vi "GCD and LCM.vi"() -> ()   [LabVIEW 2026]
panel:
  out "LCM":dbl
  out "GCD":dbl
  in  "Input Number (B)":dbl
  in  "Input Number (A)":dbl
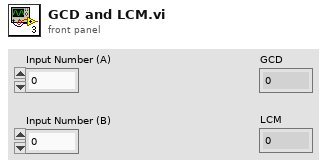
[diagram p1: front panel]
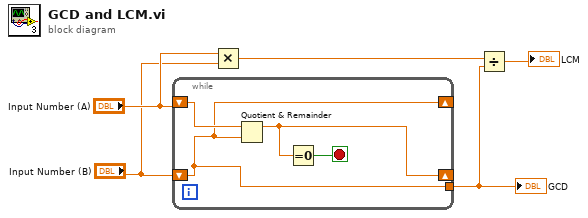
[diagram p0: block diagram]
diagram:
  n1 = while {
    shift-right: [w6] -> _
    shift-left: "Input Number (A)" -> [w9]
    shift-right: [w8] -> _
    shift-left: "Input Number (B)" -> [w6]
    tunnel: [w6] -> w1
    stop <- w7 stop-if-true
    n2 = Quotient & Remainder(x=w9, y=w6) -> (x-y*floor(x/y)=w8:dbl)  [unwired: 1 out]
    n3 = Equal To 0?(x=w8) -> (x = 0?=w7:bool)
  }
  "GCD" <- w1
  n4 = Multiply(x="Input Number (A)", y="Input Number (B)") -> (x*y=w4:dbl)
  n5 = Divide(x=w4, y=w1) -> (x/y=→"LCM":dbl)
